vi "demo1.vi"() -> ()   [LabVIEW 2020]
panel:
  out "Client served":i32
  in  "Boolean":bool
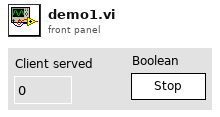
[diagram p1: front panel]
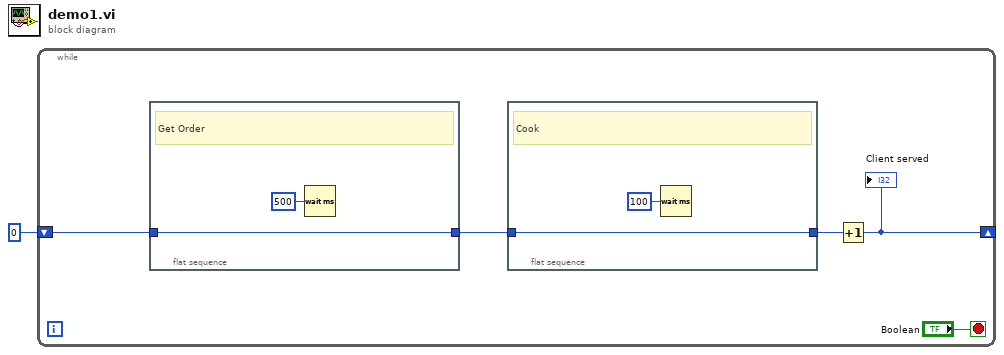
[diagram p0: block diagram]
diagram:
  n1 = while {
    shift-right: [w2] -> _
    shift-left: 0 -> [w5]
    stop <- "Boolean" stop-if-true
    n2 = flat-sequence {
      tunnel: w5 -> [w9]
      tunnel: [w9] -> w4
      frame #0 {
        # "Get Order"
        n3 = Wait (ms)(milliseconds to wait=u32 500) -> ()  [unwired: 1 out]
      }
    }
    n4 = flat-sequence {
      tunnel: w4 -> [w7]
      tunnel: [w7] -> w3
      frame #0 {
        # "Cook"
        n5 = Wait (ms)(milliseconds to wait=u32 100) -> ()  [unwired: 1 out]
      }
    }
    n6 = Increment(x=w3) -> (x+1=w2:i32)
    "Client served" <- w2
  }
